vi "Add Fixture Annotated Tool.vi"(8 "error in (no error)":errorcluster, 11 "server id":i32) -> (0 "error out":errorcluster, 3 "server id out":i32)   [LabVIEW 2020, in "MCP Server tests.lvlib"]
doc: "Test helper. Registers fake tool annotated.vi, which lies beside this VI, as an MCP tool with the title Annotated Fixture Tool and the annotations readOnlyHint true and destructiveHint false (idempotentHint and openWorldHint not set)."
uses:
  MCP Server tests.lvlib
  src/MCP Server/Tool Annotations.ctl
  src/MCP Server/Tool Hint.ctl
  src/MCP Server/MCP Server.lvlib
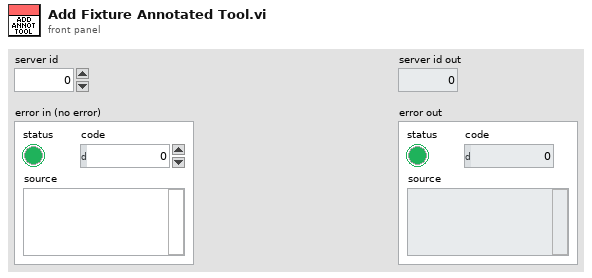
[diagram p1: front panel]
types:
  T1 = typedef "MCP Server.lvlib/Tool Annotations.ctl" = cluster{"readOnlyHint":T2, "destructiveHint":T2, "idempotentHint":T2, "openWorldHint":T2}
  T2 = typedef "MCP Server.lvlib/Tool Hint.ctl" = enum16{"not set", "true", "false"}
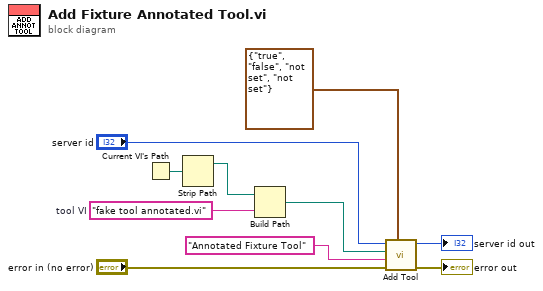
[diagram p0: block diagram]
diagram:
  w8 = "fake tool annotated.vi"  # tool VI
  n1 = Current VI's Path() -> (path=w10:path)
  n2 = Strip Path(path=w10) -> (stripped path=w9:path)  [unwired: 1 out]
  n3 = Build Path(base path=w9, name or relative path=w8) -> (appended path=w6:path)
  n4 = call "Add Tool.vi"("annotations"=T1 {"readOnlyHint"=enum."true", "destructiveHint"=enum."false", "idempotentHint"=enum."not set", "openWorldHint"=enum."not set"}, "error in (no error)"="error in (no error)", "title"="Annotated Fixture Tool", "vi path"=w6, "server id"="server id") -> ("error out"=→"error out":errorcluster, "server id out"=→"server id out":i32)  [unwired: 5 in]
